vi "Destroy User Event - Stop.vi"(8 "error in (no error)":errorcluster, 11 "Stop Event":refnum<user-event>) -> (0 "error out":errorcluster)   [LabVIEW 2021]
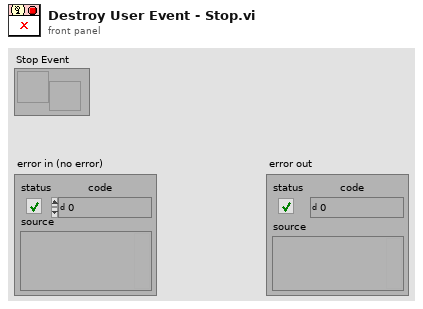
[diagram p1: front panel]
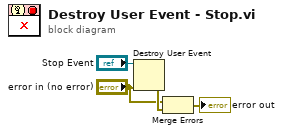
[diagram p0: block diagram]
diagram:
  n1 = Destroy User Event(user event="Stop Event", error in="error in (no error)") -> (error out=w2:errorcluster)
  n2 = Merge Errors("error in (no error)", w2) -> (→"error out":errorcluster)
